vi "Test Retry Resends Original Command.vi"(8 "error in (no error)":errorcluster) -> (0 "error out":errorcluster)   [LabVIEW 2019, in "RemoteControl.ZMQ.Tests.lvclass"]
uses:
  RemoteControl.ZMQ.Tests.lvclass
  <userlib>/LevyLab/RemoteControl/RemoteControl/RemoteControl.lvclass/RemoteControl.ctl
  <vilib>/numeric/Random Number (Range) U64.vi
  ea5dac89-44c8-4270-b814-2c06dabdc587.vi
  <vilib>/numeric/sub_Random U32.vi
  ea5dac89-44c8-4270-b814-2c06dabdc587.vi/8a413093-aa11-4f93-94f1-5b9fe02facac.vi
  ea5dac89-44c8-4270-b814-2c06dabdc587.vi/b885af2a-e049-452f-b1a7-e5e1b9c14209.vi
  <vilib>/Utility/Data Type/Get Type Information.vi
  <vilib>/JDP Science/JSONtext/JSON text to Variant.vi
  <vilib>/addons/_JKI Toolkits/Caraya/classes/Assert/Assert Equal Value_Variant.vi
  <vilib>/addons/_JKI Toolkits/Caraya/classes/Assert/Assert Greater Or Equal_Variant.vi
  <vilib>/JDP Science/JSONtext/LVClass Serializer/JSONtext LVClass Serializer.lvclass
  <userlib>/LevyLab/RemoteControl/RemoteControl/RemoteControl.lvclass
  <vilib>/addons/_JKI Toolkits/Caraya/classes/Assert/Assert.lvclass
  <vilib>/addons/_JKI Toolkits/Caraya/classes/Test/Test.lvclass
  C:/Users/patrick/Documents/GitHub/Instrument-Subsystems/RemoteControl.ZMQ/src/RemoteControl.ZMQ/RemoteControl.ZMQ.lvclass
  C:/Program Files/National Instruments/LabVIEW 2019/user.lib/LevyLab/RemoteControl/RemoteControl/RemoteControl.lvclass
  C:/Program Files/National Instruments/LabVIEW 2019/vi.lib/JKI/JKI SMO/SMO/SMO.lvclass
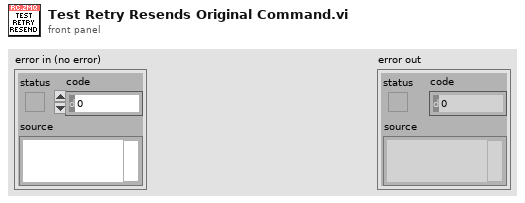
[diagram p1: front panel]
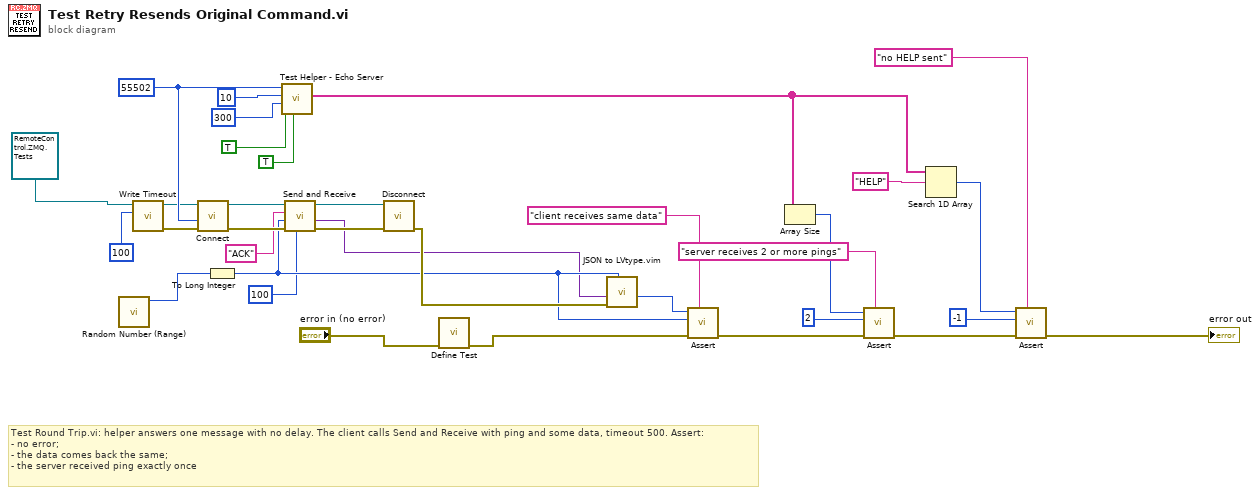
[diagram p0: block diagram]
diagram:
  w30 = u16 55502 ("Port")
  # "Test Round Trip.vi: helper answers one message with no delay. The client calls Send and Receive with ping and some data, timeout 500. Assert:\n- no error;\n- the data comes back the same;\n- the server received ping exactly once"
  n1 = call-poly <vilib>:"Random Number (Range).vi"() -> ("number"=w20:u64)  [unwired: 11 in]
  n2 = call <userlib>:"Write Timeout.vi"("timeout (ms) [500]"=100 ("timeout in ms (100)"), "RemoteControl in"=refnum<class "RemoteControl.ZMQ.Tests.lvclass"> refnum ("RemoteControl.ZMQ.Tests.lvclass")) -> ("error out"=w18:errorcluster, "RemoteControl out"=w17:refnum<class "RemoteControl.ZMQ.Tests.lvclass">)  [unwired: 8 in]
  n3 = call <userlib>:"Connect.vi"("error in (no error)"=w18, "Port"=w30, "RemoteControl in"=w17) -> ("error out"=w32:errorcluster, "RemoteControl in"=w34:refnum<class "RemoteControl.ZMQ.Tests.lvclass">)  [unwired: 7 in]
  n4 = To Long Integer(number=w20) -> (32bit integer=w15:i32)
  n5 = call "Test Helper - Echo Server.vi"("Delay 1st reply only"=TRUE, "Answer?"=TRUE, "reply delay (ms)"=u32 300, "number of messages"=10, "port"=w30) -> ("Commands"=w10:string[])  [unwired: 5 in, 1 out]
  n6 = call <userlib>:"Send and Receive.vi"("timeout (ms) [500]"=100, "error in (no error)"=w32, "Data"=w15, "Command"="ACK", "RemoteControl in"=w34) -> ("error out"=w31:errorcluster, "Data out"=w14:variant, "RemoteControl in"=w33:refnum<class "RemoteControl.ZMQ.Tests.lvclass">)  [unwired: 3 in, 1 out]
  n7 = call <userlib>:"Disconnect.vi"("error in (no error)"=w31, "RemoteControl in"=w33) -> ("error out"=w27:errorcluster)  [unwired: 8 in, 1 out]
  n8 = call <vilib>:"Define Test.vi"("error in (no error)"="error in (no error)") -> ("error out"=w4:errorcluster)  [unwired: 9 in, 1 out]
  n9 = call "JSON to LVtype.vim"("type"=w15, "error in (no error)"=w27, "JSON Data in"=w14) -> ("Data out"=w13:i32)  [unwired: 7 in, 1 out]
  n10 = call-poly <vilib>:"Assert.vi"("Label"="client receives same data", "error in (no error)"=w4, "Actual"=w15, "Expected"=w13) -> ("error out"=w24:errorcluster)  [unwired: 6 in, 1 out]
  n11 = Array Size(array=w10) -> (size(s)=w25:i32)
  n12 = call-poly <vilib>:"Assert.vi"("Label"="server receives 2 or more pings", "error in (no error)"=w24, "Actual"=2 ("size(s)"), "Expected"=w25) -> ("error out"=w11:errorcluster)  [unwired: 6 in, 1 out]
  n13 = Search 1D Array(1D array=w10, element="HELP") -> (index of element=w8:i32)  [unwired: 1 in]
  n14 = call-poly <vilib>:"Assert.vi"("Label"="no HELP sent", "error in (no error)"=w11, "Actual"=-1 ("size(s)"), "Expected"=w8) -> ("error out"=→"error out":errorcluster)  [unwired: 6 in, 1 out]
